vi "Check and Override Channel Configuration.vi"(8 "error in (no error)":errorcluster, 10 "Custom Config Data in":u8[](array[numeric]) format="%.0x", 11 "CIFFIFO in":refnum<class "CIF_CIPC_Fifo_DAQ.lvclass">) -> (0 "error out":errorcluster, 2 "Custom Config Data out":u8[](array[numeric]) format="%.0x", 3 "CIFFIFO out":refnum<class "CIF_CIPC_Fifo_DAQ.lvclass">)   [LabVIEW 2021, in "CIF_CIPC_Fifo_DAQ.lvclass"]
uses:
  CIF_CIPC_Fifo_DAQ.lvclass
  <vilib>/CIF Foundation/CIF Channels Core/ChannelCommon/ChannelCommon.lvlib
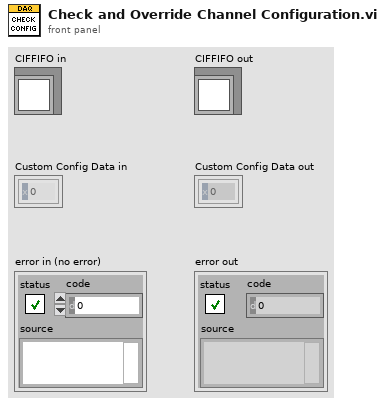
[diagram p1: front panel]
types:
  T1 = typedef "ChannelCommon.lvlib/FIFO Config.ctl" = cluster{"Max Bytes/Msg":u64, "Max Msg/FIFO":u64, "Flags":u64, "Custom Data":u8[]}
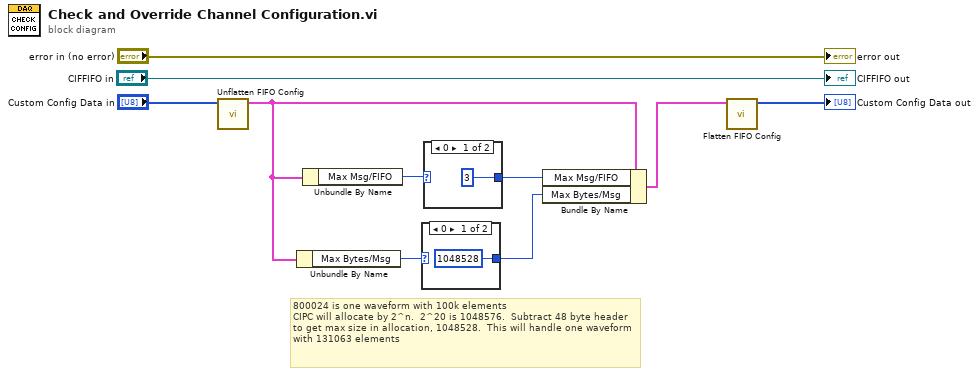
[diagram p0: block diagram]
diagram:
  # "800024 is one waveform with 100k elements\nCIPC will allocate by 2^n.  2^20 is 1048576.  Subtract 48 byte header to get max size in allocation, 1048528.  This will handle one waveform with 131063 elements"
  n1 = call <vilib>:"Unflatten FIFO Config.vi"("Flattened Data in"="Custom Config Data in") -> ("FIFO Config out"=w5:T1)  [unwired: 8 in, 2 out]
  n2 = Unbundle By Name(w5) -> ("Max Bytes/Msg"=w7:u64)
  n3 = Unbundle By Name(w5) -> ("Max Msg/FIFO"=w6:u64)
  n4 = case shown="0" w7 {
    selector: w7 -> [_ w12]
    tunnel: [u64 1048528 ("y") w12] -> w2
    frame 0 {
    }
    frame 1, Default {
    }
  }
  n5 = case shown="0" w6 {
    selector: w6 -> [_ w14]
    tunnel: [u64 3 ("y") w14] -> w3
    frame 0 {
    }
    frame 1, Default {
    }
  }
  n6 = Bundle By Name(cluster=w5, "Max Msg/FIFO"=w3, "Max Bytes/Msg"=w2) -> (w4:T1)
  n7 = call <vilib>:"Flatten FIFO Config.vi"("FIFO Config in"=w4) -> ("Flattened FIFO Config"=→"Custom Config Data out":u8[])  [unwired: 10 in]
  "error out" <- "error in (no error)"
  "CIFFIFO out" <- "CIFFIFO in"
